vi "Run Test (Object).vi"(4 "timeout (2000 ms)":i32=2000, 5 "Test Report":refnum<class "Test Report.lvclass">, 6 "Verbose":bool, 7 "Report Path":path, 8 "error in":errorcluster, 10 "Object":refnum<class>, 11 "Interactive (T)":bool=TRUE) -> (0 "error out":errorcluster, 3 "Test Results":refnum<class "Test Result.lvclass">)   [LabVIEW 2020, in "Caraya.lvlib"]
doc: "\"Run Tests\" from a class instance:\n- Dynamically discovers Caraya unit tests in a class and runs them\n- Outputs results in a UI ans/or Test Report (J-Unit or text)\n\n(Not compatible with RT targets or RunTime Engine)"
uses:
  Caraya.lvlib
  classes/Test Report/Test Report.lvclass
  classes/Test Result/Test Result.lvclass
  classes/Test Runner.Class/Test Runner.Class.lvclass
  C:/projects/caraya/src/classes/Test Runner/Test Runner.lvclass
  classes/Test Runner/Test Runner.lvclass
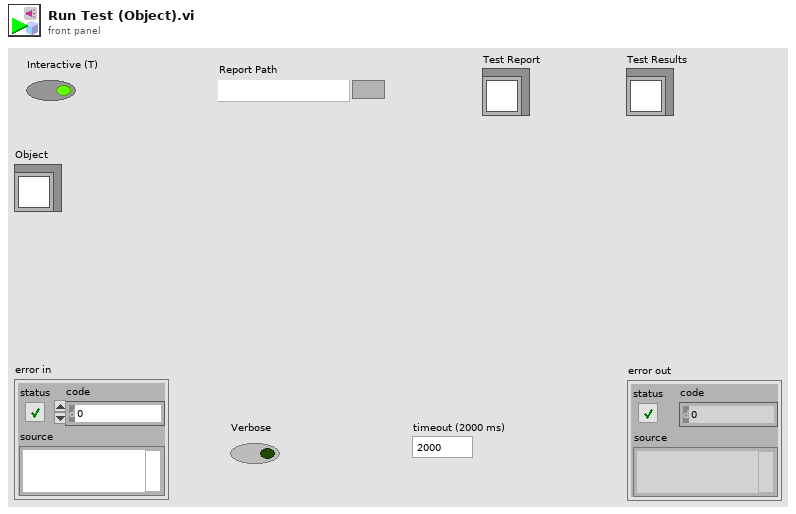
[diagram p1: front panel]
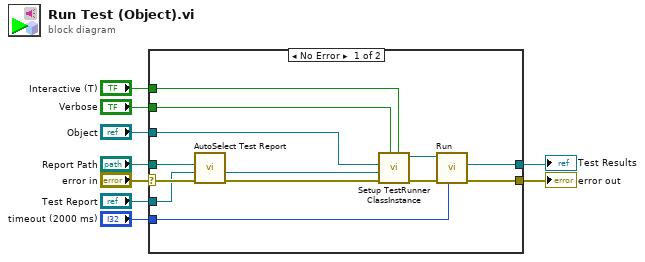
[diagram p0: block diagram]
diagram:
  n1 = case shown="No Error" "error in" {
    selector: "error in" -> [w21 w23]
    tunnel: [w22 w23] -> w9
    tunnel: "Verbose" -> [w15 _]
    tunnel: "Interactive (T)" -> [w14 _]
    tunnel: "Test Report" -> [w19 _]
    tunnel: "Object" -> [w16 _]
    tunnel: "Report Path" -> [w20 _]
    tunnel: "timeout (2000 ms)" -> [w11 _]
    tunnel: [w10 _] -> w1
    frame No Error {
      n2 = call "AutoSelect Test Report.vi"("error in (no error)"=w21, "Test Report in"=w19, "Report Path"=w20) -> ("error out"=w18:errorcluster, "Test Report out"=w17:refnum<class "Test Report.lvclass">)  [unwired: 7 in]
      n3 = call "Setup TestRunner ClassInstance.vi"("Interactive (T)"=w14, "Verbose (F)"=w15, "error in (no error)"=w18, "Test Report"=w17, "Instance"=w16) -> ("error out"=w13:errorcluster, "Test Runner.Class out"=w12:refnum<class "Test Runner.Class.lvclass">)  [unwired: 5 in]
      n4 = call "Run.vi"("timeout"=w11, "error in (no error)"=w13, "Test Runner in"=w12) -> ("error out"=w22:errorcluster, "Test Suite Results"=w10:refnum<class "Test Result.lvclass">)  [unwired: 6 in, 1 out]
    }
    frame Error {
    }
  }
  "error out" <- w9
  "Test Results" <- w1
